vi "Respawn.vi"(0 "State":T1={"Tick"=0, "Phase"=0, "PhaseTicks"=0, "Level"=1, "Room"=0, "X10"=0, "Y10"=0, "VY10"=0, "Mode"=0, "Facing"=0, "Run"=0, "Vert"=0, "StandY"=0, "EntryX10"=0, "EntryY10"=0, "EntryMode"=0, "Lives"=4, "Score"=0, "NextLife"=10000, "KeyR"=0, "KeyB"=0, "KeyY"=0, "Torch"=FALSE, "FloorPhase"=0, "Dead"=FALSE, "LevelStart"=FALSE, "Quit"=FALSE, "Sound"=0, "Seed"=12345, "DemoStep"=0, "Tiles"=[], "World"=[], "Enemies"=[], "Highscores"=[], "Name"=[0, 0, 0], "Cursor"=0}, 11 "error in":errorcluster) -> (4 "State out":T1={"Tick"=0, "Phase"=0, "PhaseTicks"=0, "Level"=1, "Room"=0, "X10"=0, "Y10"=0, "VY10"=0, "Mode"=0, "Facing"=0, "Run"=0, "Vert"=0, "StandY"=0, "EntryX10"=0, "EntryY10"=0, "EntryMode"=0, "Lives"=4, "Score"=0, "NextLife"=10000, "KeyR"=0, "KeyB"=0, "KeyY"=0, "Torch"=FALSE, "FloorPhase"=0, "Dead"=FALSE, "LevelStart"=FALSE, "Quit"=FALSE, "Sound"=0, "Seed"=12345, "DemoStep"=0, "Tiles"=[], "World"=[], "Enemies"=[], "Highscores"=[], "Name"=[0, 0, 0], "Cursor"=0}, 15 "error out":errorcluster)   [LabVIEW 2020, in "GH_Engine.lvlib"]
doc: "Puts Claude back to the arrival point of the room (after a life was lost): position and climbing mode of the arrival, standing still, enemies of the room back at their start."
uses:
  GH_Engine.lvlib
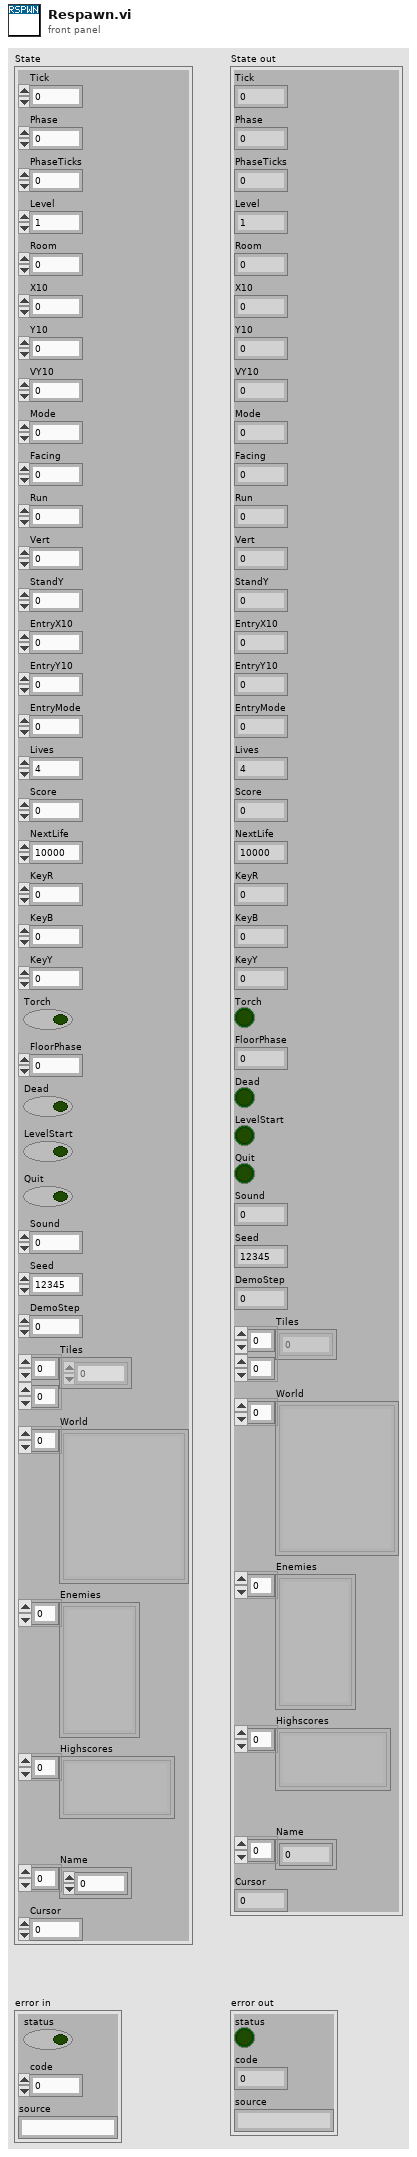
[diagram p1: front panel]
types:
  T1 = cluster{"Tick":u32, "Phase":i32, "PhaseTicks":i32, "Level":i32, "Room":i32, "X10":i32, "Y10":i32, "VY10":i32, "Mode":i32, "Facing":i32, "Run":i32, "Vert":i32, "StandY":i32, "EntryX10":i32, "EntryY10":i32, "EntryMode":i32, "Lives":i32, "Score":i32, "NextLife":i32, "KeyR":i32, "KeyB":i32, "KeyY":i32, "Torch":bool, "FloorPhase":i32, "Dead":bool, "LevelStart":bool, "Quit":bool, "Sound":i32, "Seed":u32, "DemoStep":i32, "Tiles":u8[][], "World":cluster{"ID":string, "Depth":i32, "Column":i32, "Tiles":u8[][]}[], "Enemies":cluster{"Kind":i32, "X10":i32, "Y10":i32, "Dir":i32, "Mode":i32}[], "Highscores":cluster{"Score":i32, "Name":string}[], "Name":i32[], "Cursor":i32}
  T2 = cluster{"Kind":i32, "X10":i32, "Y10":i32, "Dir":i32, "Mode":i32}[]
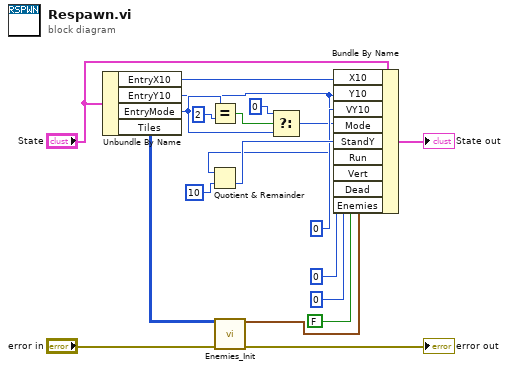
[diagram p0: block diagram]
diagram:
  n1 = Unbundle By Name("State") -> ("EntryX10"=w3:i32, "EntryY10"=w4:i32, "EntryMode"=w5:i32, "Tiles"=w6:u8[][])
  n2 = Equal?(x=w5, y=2) -> (x = y?=w10:bool)
  n3 = Quotient & Remainder(x=w4, y=10) -> (floor(x/y)=w15:i32)  [unwired: 1 out]
  n4 = call "Enemies_Init.vi"("Tiles"=w6, "error in"="error in") -> ("Enemies"=w7:T2, "error out"=→"error out":errorcluster)  [unwired: 12 in]
  n5 = Select(t=0, s=w10, f=w5) -> (s? t:f=w12:i32)
  n6 = Bundle By Name(cluster="State", "X10"=w3, "Y10"=w4, "VY10"=0, "Mode"=w12, "StandY"=w15, "Run"=0, "Vert"=0, "Dead"=FALSE, "Enemies"=w7) -> (→"State out":T1)
